vi "Import Groups.vi"(8 "error in (no error)":errorcluster, 10 "Path":path, 11 "BluelinesRedlines in":refnum<class "BluelinesRedlines.lvclass">) -> (0 "error out":errorcluster, 3 "BluelinesRedlines out":refnum<class "BluelinesRedlines.lvclass">)   [LabVIEW 2020, in "VolatusGUIElements.lvlib" / "BluelinesRedlines.lvclass"]
uses:
  BluelinesRedlines.lvclass
  BluelinesRedlines.lvclass/BluelinesRedlines.ctl
  lv-cdm/CDM-Config/Config-JSON/Config-JSON.lvclass
  lv-cdm/CDM-Config/Config Storage/Config Storage.lvclass
  lv-cdm/CDM-Config/Config Manager/Config Manager.lvclass
  lv-cdm/CDM-Config/Config Element/Config Element.lvclass
  User BluelinesRedlines/User BluelinesRedlines.lvclass
  VolatusGUI/BluelinesRedlines Source/BLRL Type.ctl
  VolatusGUI/BluelinesRedlines Source/BluelinesRedlines Source.lvclass
  VolatusErrorUtilities/MultiErrors/MultiErrors.lvclass
  C:/dev/lv20CE/relink/lv-cdm/CDM-Config/Config Storage/Config Storage.lvclass
  C:/dev/lv20CE/relink/lv-cdm/CDM-Config/Config-JSON/Config-JSON.lvclass
  C:/dev/lv20CE/relink/lv-volatus/VolatusGUIElements/User BluelinesRedlines/User BluelinesRedlines.lvclass
  C:/dev/lv20CE/relink/lv-volatus/VolatusGUI/BluelinesRedlines Source/BluelinesRedlines Source.lvclass
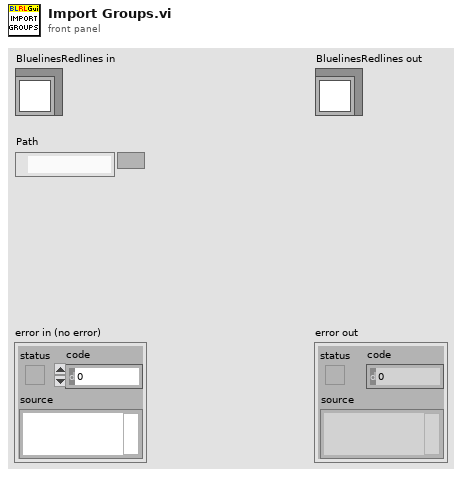
[diagram p1: front panel]
types:
  T1 = typedef "VolatusGUI.lvlib/BluelinesRedlines Source.lvclass/BLRL Type.ctl" = enum16{"Blueline", "Redline"}
  T2 = map{string, refnum<class "BluelinesRedlines Source.lvclass">}
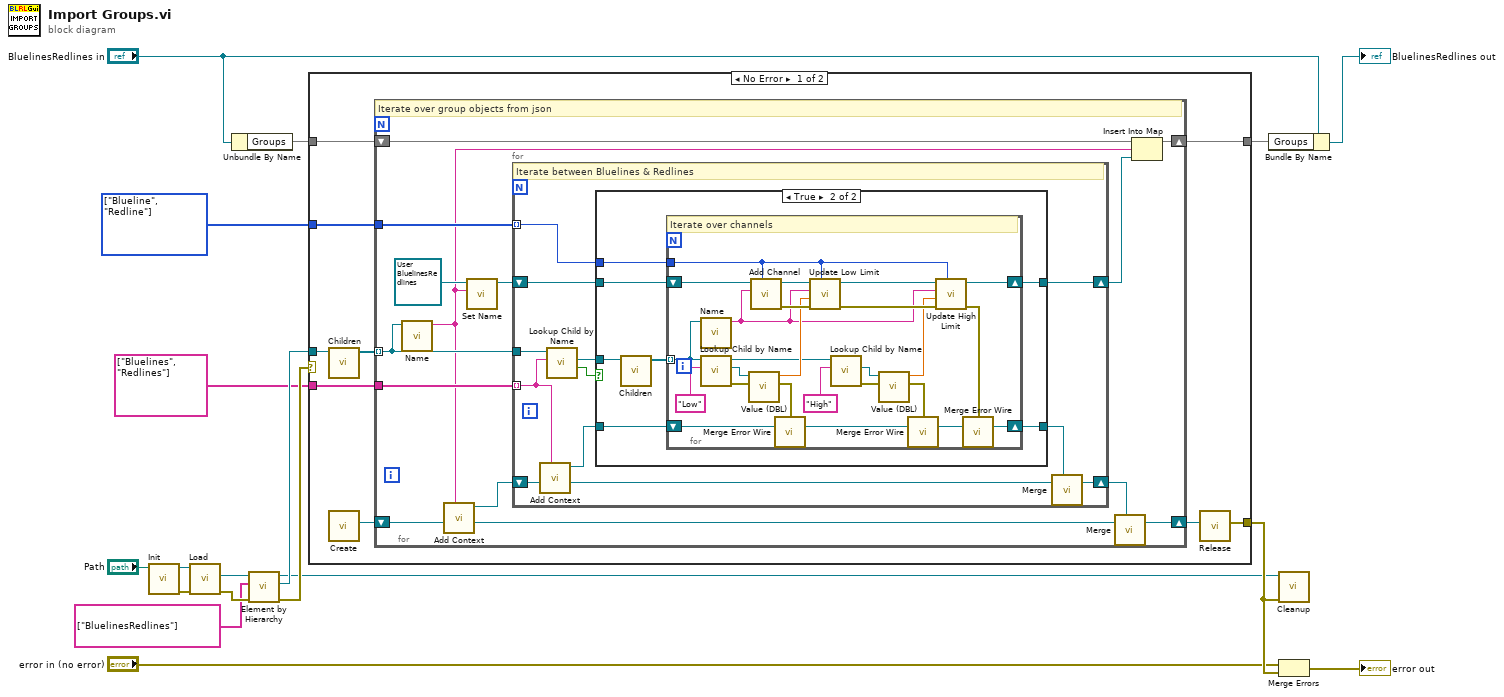
[diagram p0: block diagram]
diagram:
  w1 = T1[] [enum."Blueline", enum."Redline"] items=["Blueline", "Redline"]
  n1 = call "Init.vi"("Path"="Path") -> ("error out"=w14:errorcluster, "Config-JSON out"=w15:refnum<class "Config-JSON.lvclass">)  [unwired: 9 in]
  n2 = call "Load.vi"("error in (no error)"=w14, "Config Storage in"=w15) -> ("error out"=w12:errorcluster, "Config"=w13:refnum<class "Config Manager.lvclass">)  [unwired: 7 in, 1 out]
  n3 = Unbundle By Name("BluelinesRedlines in") -> ("Groups"=w5:T2)
  n4 = call "Element by Hierarchy.vi"("error in (no error)"=w12, "Hierarchy"=string[] ["BluelinesRedlines"], "Config Manager in"=w13) -> ("error out"=w10:errorcluster, "Config Element"=w9:refnum<class "Config Element.lvclass">, "Config Manager out"=w7:refnum<class "Config Manager.lvclass">)  [unwired: 6 in]
  n5 = case shown="No Error" w10 {
    selector: w10 -> [_ w89]
    tunnel: w9 -> [w27 _]
    tunnel: [w20 w89] -> w18
    tunnel: w5 -> [w25 w88]
    tunnel: [w19 w88] -> w3
    tunnel: string[] ["Bluelines", "Redlines"] -> [w24 _]
    tunnel: w1 -> [w23 _]
    frame No Error {
      n6 = call "Children.vi"("Config Element in"=w27) -> ("Elements"=w26:refnum<class "Config Element.lvclass">[])  [unwired: 9 in, 1 out]
      n7 = call "Create.vi"() -> ("MultiErrors out"=w22:refnum<class "MultiErrors.lvclass">)  [unwired: 11 in]
      n8 = for {
        tunnel: w26 -> [w39] mode=indexing
        shift-right: [w35] -> w19
        shift-left: w25 -> [w36]
        tunnel: w24 -> [w38]
        tunnel: w23 -> [w37]
        shift-right: [w28] -> w21
        shift-left: w22 -> [w33]
        # "Iterate over group objects from json"
        n9 = call "Name.vi"("Config Element in"=w39) -> ("Name"=w32:string)  [unwired: 9 in, 1 out]
        n10 = call "Add Context.vi"("Context"=w32, "MultiErrors in"=w33) -> ("Original Context"=w30:refnum<class "MultiErrors.lvclass">, "Added Context"=w31:refnum<class "MultiErrors.lvclass">)  [unwired: 8 in]
        n11 = call "Set Name.vi"("Name"=w32, "User BluelinesRedlines in"=refnum<class "User BluelinesRedlines.lvclass"> refnum) -> ("User BluelinesRedlines out"=w40:refnum<class "User BluelinesRedlines.lvclass">)  [unwired: 8 in, 1 out]
        n12 = for {
          shift-right: [w48] -> w34
          shift-left: w40 -> [w49]
          tunnel: w39 -> [w53]
          tunnel: w38 -> [w46] mode=indexing
          tunnel: w37 -> [w52] mode=indexing
          shift-right: [w42] -> w29
          shift-left: w31 -> [w47]
          # "Iterate between Bluelines & Redlines"
          n13 = call "Add Context.vi"("Context"=w46, "MultiErrors in"=w47) -> ("Original Context"=w44:refnum<class "MultiErrors.lvclass">, "Added Context"=w45:refnum<class "MultiErrors.lvclass">)  [unwired: 8 in]
          n14 = call "Lookup Child by Name.vi"("Name"=w46, "Config Element in"=w53) -> ("Found"=w51:bool, "Child"=w50:refnum<class "Config Element.lvclass">)  [unwired: 6 in, 2 out]
          n15 = case shown="True" w51 {
            tunnel: w52 -> [_ w59]
            tunnel: w50 -> [_ w62]
            tunnel: w49 -> [w55 w60]
            tunnel: [w55 w58] -> w48
            tunnel: w45 -> [w54 w57]
            tunnel: [w54 w56] -> w43
            frame False {
            }
            frame True {
              n16 = call "Children.vi"("Config Element in"=w62) -> ("Elements"=w61:refnum<class "Config Element.lvclass">[])  [unwired: 9 in, 1 out]
              n17 = for {
                tunnel: w61 -> [w84] mode=indexing
                shift-right: [w70] -> w58
                shift-left: w60 -> [w86]
                tunnel: w59 -> [w74]
                shift-right: [w63] -> w56
                shift-left: w57 -> [w69]
                # "Iterate over channels"
                n18 = call "Name.vi"("Config Element in"=w84) -> ("Name"=w72:string)  [unwired: 9 in, 1 out]
                n19 = call "Lookup Child by Name.vi"("Name"="Low", "Config Element in"=w84) -> ("error out"=w83:errorcluster, "Child"=w82:refnum<class "Config Element.lvclass">, "Config Element out"=w76:refnum<class "Config Element.lvclass">)  [unwired: 6 in, 1 out]
                n20 = call "Value (DBL).vi"("error in (no error)"=w83, "Config Element in"=w82) -> ("error out"=w68:errorcluster, "DBL Value"=w81:dbl)  [unwired: 8 in]
                n21 = call "Add Channel.vi"("Type"=w74, "Channel Name"=w72, "User BluelinesRedlines in"=w86) -> ("error out"=w87:errorcluster, "User BluelinesRedlines out"=w85:refnum<class "User BluelinesRedlines.lvclass">)  [unwired: 7 in]
                n22 = call "Merge Error Wire.vi"("error in (no error)"=w68, "MultiErrors in"=w69) -> ("MultiErrors out"=w67:refnum<class "MultiErrors.lvclass">)  [unwired: 13 in]
                n23 = call "Update Low Limit.vi"("Type"=w74, "error in (no error)"=w87, "Low Limit"=w81, "Channel Name"=w72, "User BluelinesRedlines in"=w85) -> ("error out"=w73:errorcluster, "User BluelinesRedlines out"=w75:refnum<class "User BluelinesRedlines.lvclass">)  [unwired: 5 in]
                n24 = call "Lookup Child by Name.vi"("Name"="High", "Config Element in"=w76) -> ("error out"=w77:errorcluster, "Child"=w78:refnum<class "Config Element.lvclass">)  [unwired: 6 in, 2 out]
                n25 = call "Value (DBL).vi"("error in (no error)"=w77, "Config Element in"=w78) -> ("error out"=w66:errorcluster, "DBL Value"=w71:dbl)  [unwired: 8 in]
                n26 = call "Merge Error Wire.vi"("error in (no error)"=w66, "MultiErrors in"=w67) -> ("MultiErrors out"=w65:refnum<class "MultiErrors.lvclass">)  [unwired: 13 in]
                n27 = call "Update High Limit.vi"("Type"=w74, "error in (no error)"=w73, "High Limit"=w71, "Channel Name"=w72, "User BluelinesRedlines in"=w75) -> ("error out"=w64:errorcluster, "User BluelinesRedlines out"=w70:refnum<class "User BluelinesRedlines.lvclass">)  [unwired: 5 in]
                n28 = call "Merge Error Wire.vi"("error in (no error)"=w64, "MultiErrors in"=w65) -> ("MultiErrors out"=w63:refnum<class "MultiErrors.lvclass">)  [unwired: 13 in]
              }
            }
          }
          n29 = call "Merge.vi"("First Error In"=w44, "Second Error In"=w43) -> ("MultiErrors out"=w42:refnum<class "MultiErrors.lvclass">)  [unwired: 5 in]
        }
        n30 = call "Merge.vi"("First Error In"=w30, "Second Error In"=w29) -> ("MultiErrors out"=w28:refnum<class "MultiErrors.lvclass">)  [unwired: 5 in]
        n31 = Insert Into Map(map in=w36, key=w32, value=w34) -> (map out=w35:T2)  [unwired: 2 out]
      }
      n32 = call "Release.vi"("MultiErrors in"=w21) -> ("error out"=w20:errorcluster)  [unwired: 10 in]
    }
    frame Error {
    }
  }
  n33 = Bundle By Name(cluster="BluelinesRedlines in", "Groups"=w3) -> (→"BluelinesRedlines out":refnum<class "BluelinesRedlines.lvclass">)
  n34 = call "Cleanup.vi"("error in (no error)"=w18, "Config Manager in"=w7) -> ()  [unwired: 9 in, 1 out]
  n35 = Merge Errors("error in (no error)", w18) -> (→"error out":errorcluster)
